vi "Null Id For Parse Error.vi"(8 "error in":errorcluster, 11 "response":string) -> (0 "error out":errorcluster, 3 "response out":string)   [LabVIEW 2020, in "MCP Server.lvlib"]
doc: "A parse error (-32700) means the message could not be read, so its id is unknown: JSON-RPC asks for id null in that answer. This VI sets the id of a -32700 response to null and passes every other response through."
uses:
  MCP Server.lvlib
  <vilib>/JDP Science/JSONtext/Next JSON Value.vi
  <vilib>/JDP Science/JSONtext/String Subset.vi
  <vilib>/JDP Science/JSONtext/Parsing/Advance past next JSON Value (inlined COPY).vi
  <vilib>/JDP Science/JSONtext/Parsing/Advance past whitespace.vi
  <vilib>/JDP Science/JSONtext/Parsing/Advance past String.vi
  <vilib>/JDP Science/JSONtext/Parsing/Advance past Number.vi
  <vilib>/JDP Science/JSONtext/Parsing/Advance past Line Ending.vi
  <vilib>/JDP Science/JSONtext/Parsing/Parse Full Path or Item Name.vi
  <vilib>/JDP Science/JSONtext/Parsing/Advance past Array.vi
  <vilib>/JDP Science/JSONtext/Parsing/Advance past Object.vi
  <vilib>/JDP Science/JSONtext/support/Error Cluster From Code.vi
  <vilib>/JDP Science/JSONtext/Offset/Find Item Locations by Path.vi
  <vilib>/JDP Science/JSONtext/JSONtext.lvlib
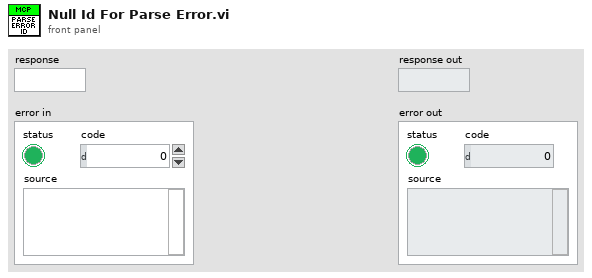
[diagram p1: front panel]
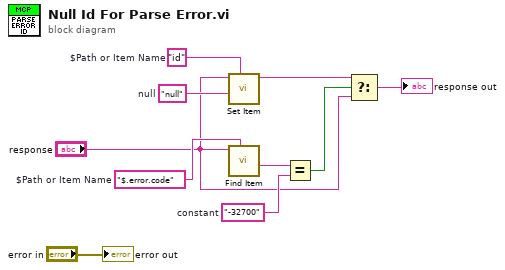
[diagram p0: block diagram]
diagram:
  w7 = "id"  # $Path or Item Name
  w6 = "null"  # null
  w8 = "-32700"  # constant
  w10 = "$.error.code"  # $Path or Item Name
  n1 = call <vilib>:"Set Item.vi"("$Path or Item Name"=w7, "JSON to Insert"=w6, "JSON"="response") -> ("<JSON>"=w5:string)  [unwired: 5 in, 2 out]
  n2 = call <vilib>:"Find Item.vi"("$Path or Item Name"=w10, "JSON"="response") -> ("<JSON>"=w9:string)  [unwired: 6 in, 3 out]
  n3 = Equal?(x=w9, y=w8) -> (x = y?=w4:bool)
  n4 = Select(t=w5, s=w4, f="response") -> (s? t:f=→"response out":string)
  "error out" <- "error in"
